vi "Edit Plugin Data File.vi"(0 "configuration":T1, 5 "plugin data file path":path, 11 "error in":errorcluster) -> (15 "error out":errorcluster)   [LabVIEW 2021, in "InstrumentStudio Plug-In Editor.lvlib"]
uses:
  InstrumentStudio Plug-In Editor.lvlib
  Plugin Configuration.ctl
  <vilib>/xml/Load XML String.vi
  <vilib>/xml/Close Reference(Node).vi
  <vilib>/xml/NI_XML.lvlib
  <resource>/objmgr/DOMUserDefRef.rc
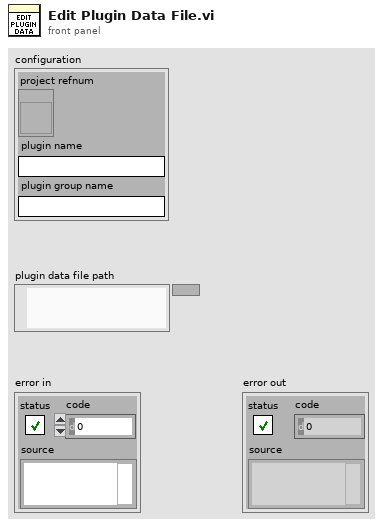
[diagram p1: front panel]
types:
  T1 = typedef "InstrumentStudio Plug-In Editor.lvlib/Plugin Configuration.ctl" = cluster{"project refnum":refnum<vi>, "plugin name":string, "plugin group name":string}
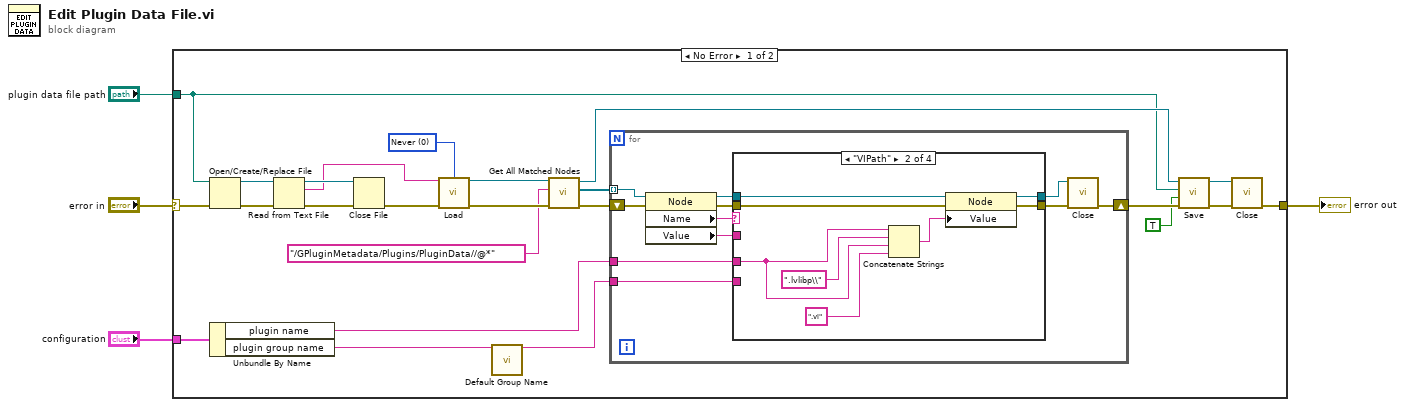
[diagram p0: block diagram]
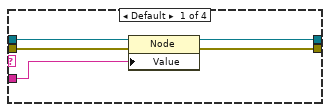
[diagram p2: hidden frame]
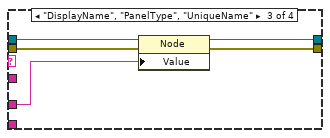
[diagram p3: hidden frame]
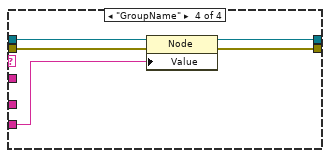
[diagram p4: hidden frame]
diagram:
  n1 = case shown="No Error" "error in" {
    selector: "error in" -> [w17 w63]
    tunnel: [w6 w63] -> w1
    tunnel: "plugin data file path" -> [w13 _]
    tunnel: "configuration" -> [w24 _]
    frame No Error {
      w10 = 0 items=["Never", "Always", "Auto"] ("validate on load (Auto)")
      n2 = Open/Create/Replace File(file path (use dialog)=w13, error in=w17) -> (refnum out=w28:refnum<file>, error out=w16:errorcluster)  [unwired: 4 in, 1 out]
      n3 = Unbundle By Name(w24) -> ("plugin name"=w23:string, "plugin group name"=w9:string)
      n4 = Read from Text File(file (use dialog)=w28, error in=w16) -> (refnum out=w27:refnum<file>, text=w11:string, error out=w15:errorcluster)  [unwired: 2 in, 1 out]
      n5 = Close File(refnum=w27, error in=w15) -> (error out=w14:errorcluster)  [unwired: 1 out]
      n6 = call-poly <vilib>:"Load.vi"("XML string"=w11, "validate on load (Auto)"=w10, "error in (no error)"=w14) -> ("DOM document out"=w12:refnum<k20>, "error out"=w20:errorcluster)  [unwired: 10 in, 1 out]
      n7 = call "Default Group Name.vi"("group name in"=w9) -> ("group name out"=w22:string)  [unwired: 14 in]
      n8 = call <vilib>:"Get All Matched Nodes.vi"("error in (no error)"=w20, "XPath expression"="/GPluginMetadata/Plugins/PluginData//@*", "node in"=w12) -> ("error out"=w19:errorcluster, "node result array"=w21:refnum<k20>[], "node out"=w26:refnum<k20>)  [unwired: 6 in]
      n9 = for {
        tunnel: w21 -> [w39] mode=indexing
        tunnel: w23 -> [w35]
        tunnel: w22 -> [w34]
        shift-right: [w29] -> w18
        shift-left: w19 -> [w32]
        n10 = property class="Node"(reference=w39, error in=w32) -> (reference out=w38:refnum<k20>, error out=w31:errorcluster, "Name"=w36:string, "Value"=w33:string)
        n11 = case shown="\"VIPath\"" w36 {
          tunnel: w38 -> [w44 w52 w57 w62]
          tunnel: [w43 w51 w56 w58] -> w37
          tunnel: [w42 w48 w55 w59] -> w30
          tunnel: w35 -> [_ w47 w54 _]
          tunnel: w34 -> [_ _ _ w61]
          tunnel: w33 -> [w41 _ _ _]
          tunnel: w31 -> [w40 w49 w53 w60]
          frame Default {
            n12 = property class="Node"(reference=w44, error in=w40, "Value"=w41) -> (reference out=w43:refnum<k20>, error out=w42:errorcluster)
          }
          frame "VIPath" {
            n13 = Concatenate Strings(w47, ".lvlibp\\" ("string"), w47, ".vi" ("string")) -> (w46:string)
            n14 = property class="Node"(reference=w52, error in=w49, "Value"=w46) -> (reference out=w51:refnum<k20>, error out=w48:errorcluster)
          }
          frame "DisplayName", "PanelType", "UniqueName" {
            n15 = property class="Node"(reference=w57, error in=w53, "Value"=w54) -> (reference out=w56:refnum<k20>, error out=w55:errorcluster)
          }
          frame "GroupName" {
            n16 = property class="Node"(reference=w62, error in=w60, "Value"=w61) -> (reference out=w58:refnum<k20>, error out=w59:errorcluster)
          }
        }
        n17 = call-poly <vilib>:"Close.vi"("error in (no error)"=w30, "node"=w37) -> ("error out"=w29:errorcluster)  [unwired: 7 in]
      }
      n18 = call <vilib>:"Save.vi"("error in (no error)"=w18, "overwrite file (True)"=TRUE, "XML file path"=w13, "DOM document in"=w26) -> ("error out"=w25:errorcluster, "DOM document out"=w5:refnum<k20>)  [unwired: 5 in, 1 out]
      n19 = call-poly <vilib>:"Close.vi"("error in (no error)"=w25, "node"=w5) -> ("error out"=w6:errorcluster)  [unwired: 7 in]
    }
    frame Error {
    }
  }
  "error out" <- w1
